vi "DeleteObject Wrapper Template.vi"(0 "ho":u64, 11 "error in":errorcluster) -> (4 "return value":i32, 15 "error out":errorcluster)   [LabVIEW 2020]
doc: "Deletes a GDI object (bitmap, pen, brush ...) through gdi32.dll DeleteObject (stdcall, called in any thread). It must not be selected into a device context. return value is non-zero on success. When error in carries an error the DLL is not called. Generated by tools\\Build Win32 Wrappers.vi - do not edit by hand, rebuild it."
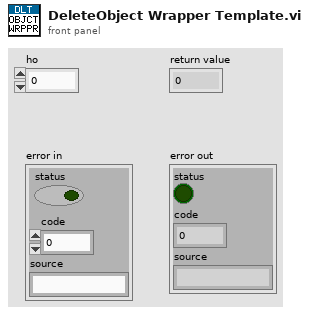
[diagram p1: front panel]
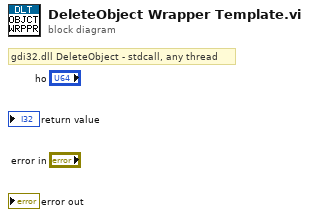
[diagram p0: block diagram]
diagram:
  # "gdi32.dll DeleteObject - stdcall, any thread"
